vi "Output Parameter Cluster Documentation--constant.vi"() -> (3 "Output Parameter Cluster Documentation":string)   [LabVIEW 2026]
doc: "This constant defines the documentation string of output parameter clusters (as a format string)."
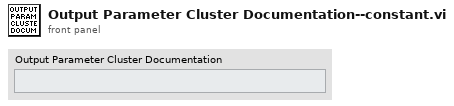
[diagram p1: front panel]
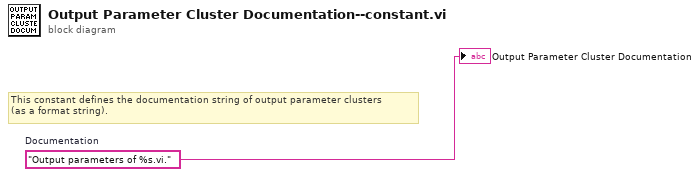
[diagram p0: block diagram]
diagram:
  w1 = "Output parameters of %s.vi."  # Documentation
  # "This constant defines the documentation string of output parameter clusters \n(as a format string)."
  "Output Parameter Cluster Documentation" <- w1
